vi "VM Spy - Dialog - Set Variable Value.vi"(6 "refresh writer ID":bool, 8 "writer ID in":u32, 9 "Display params":T1={"Num Format"=0, "Num Precision"=3, "Num Show I32"=FALSE, "Str Style"=0, "Str Wrap"=TRUE}, 10 "var name":string, 11 "VC Handle":T2=-1) -> (0 "Assigned":bool)   [LabVIEW 2021]
doc: "::: CalcExpress Toolkit :::\nCopyright (c) 2000-2026 Konstantin Shifershteyn. All rights reserved."
uses:
  vi.lib/addons/CalcExpress/cetypes.llb/VarMan Variable Context Handle.ctl
  <vilib>/Utility/miscctls.llb/LVKeyTypeDef.ctl
panel:
  in  "writer ID":u32
  in  "EnaWrap":bool=TRUE caption="Wrap"
  in  "int32":i32 caption="Int32" format="%.0x"
  in  "ShowInt32":bool caption="show I32"
  in  "IR":cluster{"Initial index":i32, "Final index":i32} caption="Index Range" {"Final index" min=0; "Initial index" min=0}
  in  "Format":u8(ring) items=["Floating point", "Scientific", "Engineering", "Binary", "Octal", "Hexadecimal", "Relative time", "Absolute time"]
  in  "prec":u8=2
  in  "a2str":string[][](array[string]) caption="Value"
  in  "a1str":string[](array[string]) caption="Value"
  in  "a2cdb":cdb[][](array[numeric]) caption="Value" format="%.2f"
  in  "a1cdb":cdb[](array[numeric]) caption="Value" format="%.2f"
  in  "cancel":bool
  in  "assign":bool
  in  "close":bool=TRUE caption="close window after assignment"
  in  "any":string
  in  "a2dbl":dbl[][](array[numeric]) caption="Value" format="%.2f"
  in  "cdb":cdb caption="Value" format="%.2f"
  in  "a1dbl":dbl[](array[numeric]) caption="Value" format="%.2f"
  in  "Display style":u32(ring) items=["Normal", "'\\' Code", "Password", "Hex dump"]
  in  "dbl":dbl caption="Value" format="%.3f"
  out "Context":string
  out "Variable":string
  in  "str":string caption="Value"
  # ":"
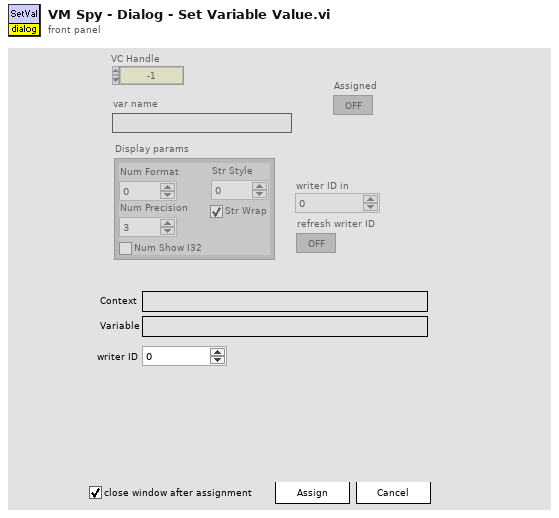
[diagram p1: front panel]
types:
  T1 = cluster{"Num Format":u32, "Num Precision":u32, "Num Show I32":bool, "Str Style":u32, "Str Wrap":bool}
  T2 = typedef "VarMan Variable Context Handle.ctl" = i32
  T3 = typedef "LVKeyTypeDef.ctl" = cluster{"Focus":bool, "Control":bool, "Shift":bool, "Key":string}
  T4 = enum32{"invalid app kind", "Development System", "Run Time System", "Student Edition", "Embedded LabVIEW", "Evaluation", "Custom"}
  T5 = typedef "eventvkey.ctl" = enum16{"ASCII", "Enter", "Return", "Shift", "Ctrl", "Alt", "Cmd", "Opt", "Caps", "NumLock", "Clear", "Break", "Up", "Down", "Left", "Right", "Insert", "Delete", "Home", "End", "PageUp", "PageDown", "Escape", "Help", "Pause", "ScrollLock", "F1", "F2", "F3", "F4", "F5", "F6", "F7", "F8", "F9", "F10", "F11", "F12", "F13", "F14", "F15", "F16", "F17", "F18", "F19", "F20", "F21", "F22", "F23", "F24", "Play", "VolumeUp", "VolumeDown", "Mute", "Two Byte Char"}
  T6 = cluster{"Shift":bool, "Ctrl":bool, "Alt":bool, "Cmd":bool, "Opt":bool}
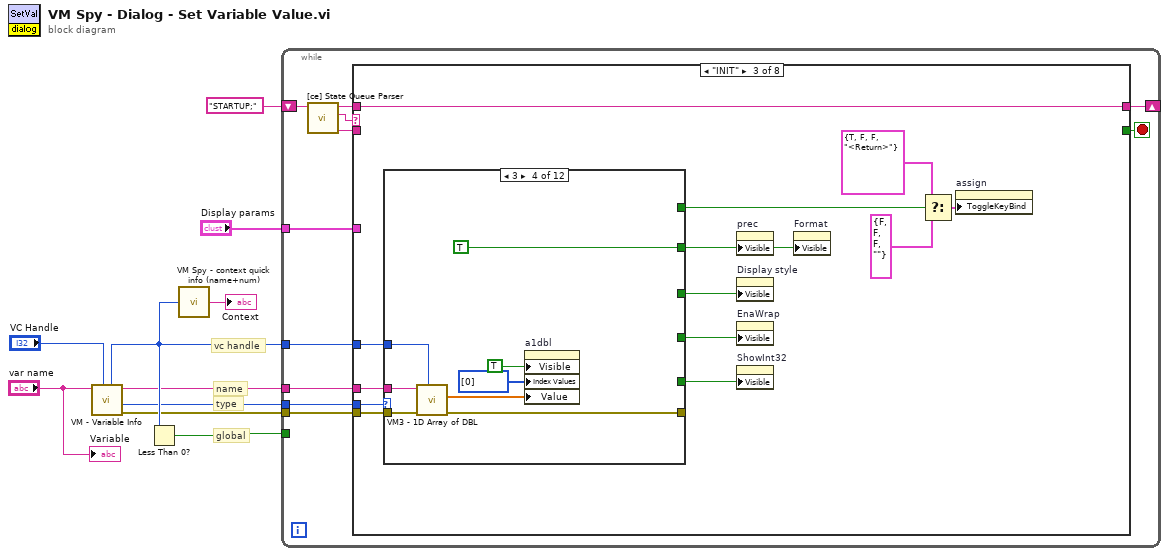
[diagram p0: block diagram]
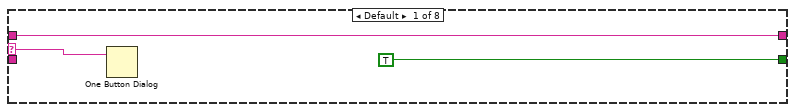
[diagram p2: hidden frame]
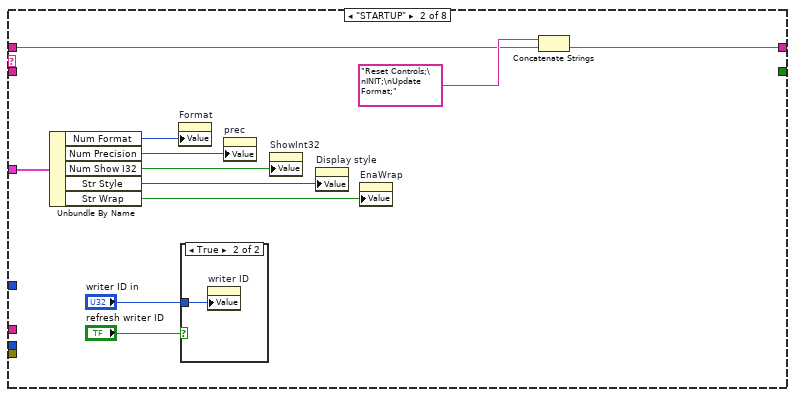
[diagram p3: hidden frame]
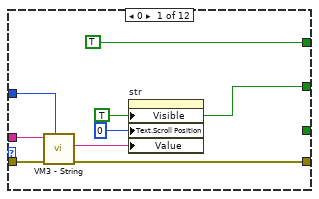
[diagram p5: hidden frame]
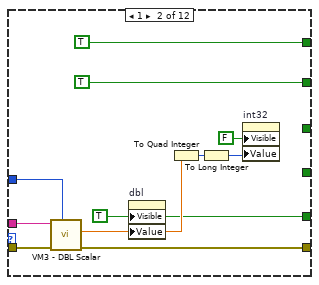
[diagram p6: hidden frame]
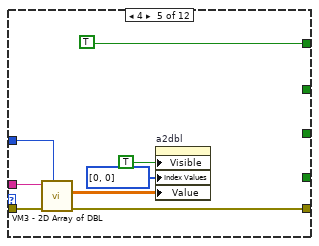
[diagram p8: hidden frame]
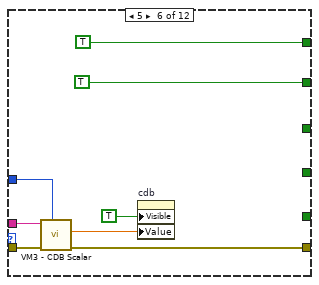
[diagram p9: hidden frame]
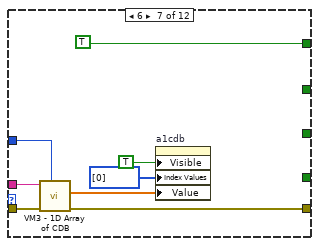
[diagram p10: hidden frame]
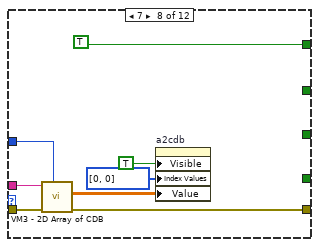
[diagram p11: hidden frame]
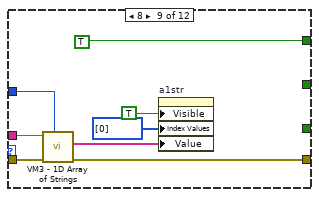
[diagram p12: hidden frame]
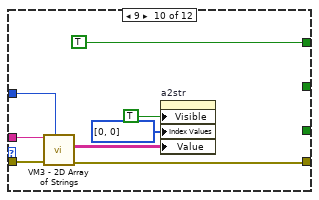
[diagram p13: hidden frame]
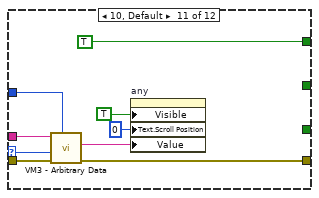
[diagram p14: hidden frame]
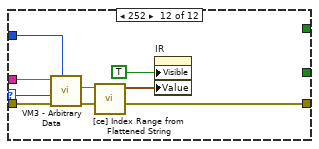
[diagram p15: hidden frame]
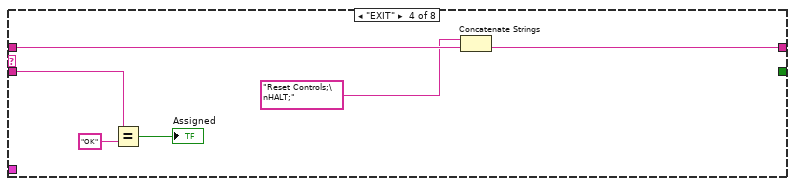
[diagram p16: hidden frame]
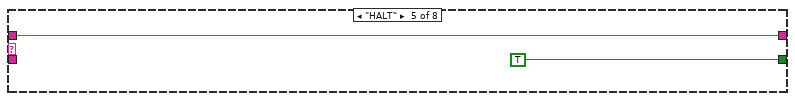
[diagram p17: hidden frame]
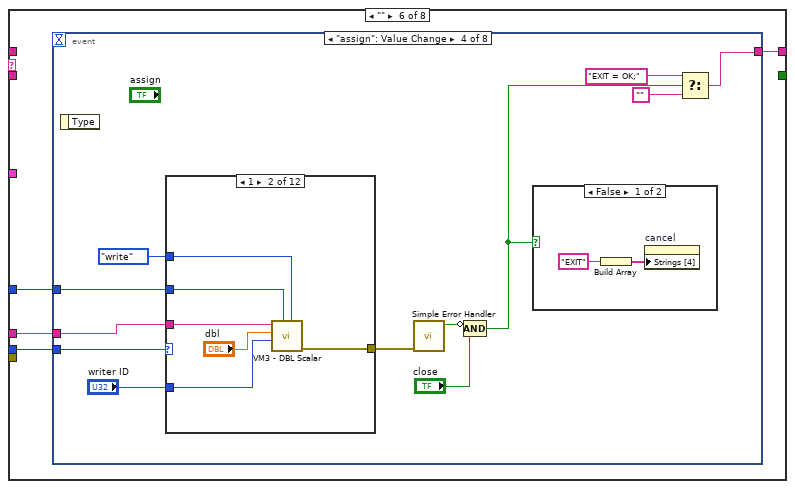
[diagram p18: hidden frame]
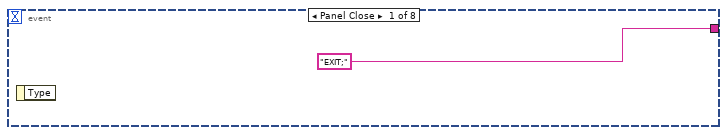
[diagram p19: hidden frame]
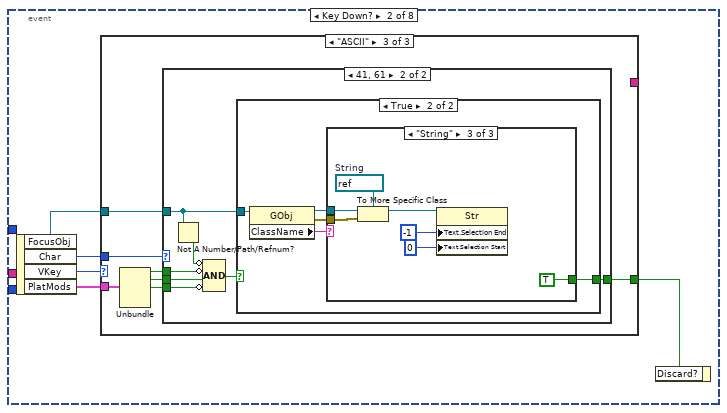
[diagram p20: hidden frame]
diagram:
  # "name"
  # "vc handle"
  # "type"
  # "global"
  n1 = call "VM - Variable Info.vi"("VC Handle"="VC Handle", "name_spec"="var name") -> ("error out"=w2:errorcluster, "var type"=w5:u32, "var name"=w7:string, "var VC Handle"=w8:T2)  [unwired: 4 in, 2 out]
  n2 = Less Than 0?(x=w8) -> (x < 0?=w6:bool)
  n3 = call "VM Spy - context quick info (name+num).vi"("handle"=w8) -> ("context info"=→"Context":string)  [unwired: 4 in]
  n4 = while {
    tunnel: w8 -> [w20]
    tunnel: w7 -> [w19]
    tunnel: w6 -> [_]
    tunnel: w5 -> [w18]
    shift-right: [w15] -> _
    shift-left: "STARTUP;" -> [w17]
    tunnel: w2 -> [w13]
    tunnel: "Display params" -> [w11]
    stop <- w21 stop-if-true
    n5 = call "[ce] State Queue Parser.vi"("input queue"=w17) -> ("state parameters"=w12:string, "state"=w16:string, "remained queue"=w14:string)  [unwired: 6 in]
    n6 = case shown="\"INIT\"" w16 {
      selector: w16 -> [w23 _ _ _ _ _ _ _]
      tunnel: [TRUE _ _ _ TRUE _ _ _] -> w21
      tunnel: w20 -> [_ _ w43 _ _ w154 _ _]
      tunnel: w19 -> [_ _ w42 _ _ w153 _ _]
      tunnel: w18 -> [_ _ w40 _ _ w152 _ w325]
      tunnel: [w24 w33 w39 w147 w150 w151 w317 w329] -> w15
      tunnel: w14 -> [w24 w34 w39 w148 w150 _ w317 w329]
      tunnel: w13 -> [_ _ w41 _ _ _ _ _]
      tunnel: w12 -> [_ _ _ w145 _ _ _ _]
      tunnel: w11 -> [_ w32 _ _ _ _ _ _]
      frame Default {
        n7 = One Button Dialog(message=w23) -> ()  [unwired: 1 in, 1 out]
      }
      frame "STARTUP" {
        n8 = Unbundle By Name(w32) -> ("Num Format"=w31:u32, "Num Precision"=w30:u32, "Num Show I32"=w29:bool, "Str Style"=w28:u32, "Str Wrap"=w27:bool)
        n9 = property on="Format" class="Ring (strict)"("Value"=w31) -> ()  [unwired: 2 in, 2 out]
        n10 = case shown="True" "refresh writer ID" {
          tunnel: "writer ID in" -> [_ w36]
          frame False {
          }
          frame True {
            n11 = property on="writer ID" class="DigNum (strict)"("Value"=w36) -> ()  [unwired: 2 in, 2 out]
          }
        }
        n12 = property on="prec" class="DigNum (strict)"("Value"=w30) -> ()  [unwired: 2 in, 2 out]
        n13 = property on="ShowInt32" class="Bool (strict)"("Value"=w29) -> ()  [unwired: 2 in, 2 out]
        n14 = property on="Display style" class="Ring (strict)"("Value"=w28) -> ()  [unwired: 2 in, 2 out]
        n15 = property on="EnaWrap" class="Bool (strict)"("Value"=w27) -> ()  [unwired: 2 in, 2 out]
        n16 = Concatenate Strings("Reset Controls;\nINIT;\nUpdate Format;" ("string"), w34) -> (w33:string)
      }
      frame "INIT" {
        n17 = case shown="3" w40 {
          selector: w40 -> [_ _ _ _ _ _ _ _ _ _ w130 w138]
          tunnel: w41 -> [w57 w67 w69 w76 w84 w92 w100 w108 w116 w124 w134 w142]
          tunnel: w42 -> [w56 w68 _ w77 w85 w93 w101 w109 w117 w125 w132 w140]
          tunnel: w43 -> [w54 w65 _ w74 w82 w90 w98 w106 w114 w122 w131 w139]
          tunnel: [w55 w66 w69 w75 w83 w91 w99 w107 w115 w123 w133 w141] -> _
          tunnel: [TRUE _ _ _ _ _ _ _ TRUE TRUE TRUE _] -> w49
          tunnel: [_ TRUE _ TRUE TRUE TRUE TRUE TRUE _ _ _ _] -> w48
          tunnel: [_ TRUE _ _ _ TRUE _ _ _ _ _ _] -> w44
          tunnel: [_ w59 _ _ _ _ _ _ _ _ _ _] -> w38
          tunnel: [w50 _ _ _ _ _ _ _ _ _ _ _] -> w37
          frame 0 {
            w50 = TRUE
            n18 = call "VM3 - String.vi"("VC Handle"=w54, "error in"=w57, "name_spec"=w56) -> ("error out"=w55:errorcluster, "value out"=w51:string)  [unwired: 5 in, 2 out]
            n19 = property on="str" class="Str"("Visible"=w50, "Text.Scroll Position"=u32 0, "Value"=w51) -> ()  [unwired: 2 in, 2 out]
          }
          frame 1 {
            w59 = TRUE
            n20 = call "VM3 - DBL Scalar.vi"("VC Handle"=w65, "error in"=w67, "name_spec"=w68) -> ("error out"=w66:errorcluster, "value out"=w62:dbl)  [unwired: 5 in, 2 out]
            n21 = property on="dbl" class="DigNum (strict)"("Visible"=w59, "Value"=w62) -> ()  [unwired: 2 in, 2 out]
            n22 = To Quad Integer(1:w62) -> (0:w61:i64)
            n23 = To Long Integer(number=w61) -> (32bit integer=w60:i32)
            n24 = property on="int32" class="DigNum (strict)"("Visible"=FALSE, "Value"=w60) -> ()  [unwired: 2 in, 2 out]
          }
          frame 2 {
          }
          frame 3 {
            n25 = call "VM3 - 1D Array of DBL.vi"("VC Handle"=w74, "error in"=w76, "name_spec"=w77) -> ("error out"=w75:errorcluster, "value out"=w70:dbl[])  [unwired: 5 in, 2 out]
            n26 = property on="a1dbl" class="Arr (strict)"("Visible"=TRUE, "Index Values"=u32[] [0], "Value"=w70) -> ()  [unwired: 2 in, 2 out]
          }
          frame 4 {
            n27 = call "VM3 - 2D Array of DBL.vi"("VC Handle"=w82, "error in"=w84, "name_spec"=w85) -> ("error out"=w83:errorcluster, "value out"=w78:dbl[][])  [unwired: 5 in, 2 out]
            n28 = property on="a2dbl" class="Arr (strict)"("Visible"=TRUE, "Index Values"=u32[] [0, 0], "Value"=w78) -> ()  [unwired: 2 in, 2 out]
          }
          frame 5 {
            n29 = call "VM3 - CDB Scalar.vi"("VC Handle"=w90, "error in"=w92, "name_spec"=w93) -> ("error out"=w91:errorcluster, "value out"=w86:cdb)  [unwired: 5 in, 2 out]
            n30 = property on="cdb" class="DigNum (strict)"("Visible"=TRUE, "Value"=w86) -> ()  [unwired: 2 in, 2 out]
          }
          frame 6 {
            n31 = call "VM3 - 1D Array of CDB.vi"("VC Handle"=w98, "error in"=w100, "name_spec"=w101) -> ("error out"=w99:errorcluster, "value out"=w94:cdb[])  [unwired: 5 in, 2 out]
            n32 = property on="a1cdb" class="Arr (strict)"("Visible"=TRUE, "Index Values"=u32[] [0], "Value"=w94) -> ()  [unwired: 2 in, 2 out]
          }
          frame 7 {
            n33 = call "VM3 - 2D Array of CDB.vi"("VC Handle"=w106, "error in"=w108, "name_spec"=w109) -> ("error out"=w107:errorcluster, "value out"=w102:cdb[][])  [unwired: 5 in, 2 out]
            n34 = property on="a2cdb" class="Arr (strict)"("Visible"=TRUE, "Index Values"=u32[] [0, 0], "Value"=w102) -> ()  [unwired: 2 in, 2 out]
          }
          frame 8 {
            n35 = call "VM3 - 1D Array of Strings.vi"("VC Handle"=w114, "error in"=w116, "name_spec"=w117) -> ("error out"=w115:errorcluster, "value out"=w110:string[])  [unwired: 5 in, 2 out]
            n36 = property on="a1str" class="Arr (strict)"("Visible"=TRUE, "Index Values"=u32[] [0], "Value"=w110) -> ()  [unwired: 2 in, 2 out]
          }
          frame 9 {
            n37 = call "VM3 - 2D Array of Strings.vi"("VC Handle"=w122, "error in"=w124, "name_spec"=w125) -> ("error out"=w123:errorcluster, "value out"=w118:string[][])  [unwired: 5 in, 2 out]
            n38 = property on="a2str" class="Arr (strict)"("Visible"=TRUE, "Index Values"=u32[] [0, 0], "Value"=w118) -> ()  [unwired: 2 in, 2 out]
          }
          frame 10, Default {
            n39 = call "VM3 - Arbitrary Data.vi"("var type in"=w130, "VC Handle"=w131, "error in"=w134, "name_spec"=w132) -> ("error out"=w133:errorcluster, "flattened value out"=w126:string)  [unwired: 3 in, 3 out]
            n40 = property on="any" class="Str"("Visible"=TRUE, "Text.Scroll Position"=u32 0, "Value"=w126) -> ()  [unwired: 2 in, 2 out]
          }
          frame 252 {
            n41 = call "VM3 - Arbitrary Data.vi"("var type in"=w138, "VC Handle"=w139, "error in"=w142, "name_spec"=w140) -> ("error out"=w141:errorcluster, "flattened value out"=w137:string)  [unwired: 3 in, 3 out]
            n42 = call "[ce] Index Range from Flattened String.vi"("Flattened string"=w137) -> ("Index Range"=w135:cluster{"Initial index":i32, "Final index":i32})  [unwired: 10 in]
            n43 = property on="IR" class="Clust (strict)"("Visible"=TRUE, "Value"=w135) -> ()  [unwired: 2 in, 2 out]
          }
        }
        n44 = property on="prec" class="DigNum (strict)"("Visible"=w48) -> ()  [unwired: 2 in, 2 out]
        n45 = property on="Display style" class="Ring (strict)"("Visible"=w49) -> ()  [unwired: 2 in, 2 out]
        n46 = property on="EnaWrap" class="Bool (strict)"("Visible"=w37) -> ()  [unwired: 2 in, 2 out]
        n47 = property on="ShowInt32" class="Bool (strict)"("Visible"=w38) -> ()  [unwired: 2 in, 2 out]
        n48 = property on="Format" class="Ring (strict)"("Visible"=w48) -> ()  [unwired: 2 in, 2 out]
        n49 = Select(t=T3 {"Focus"=TRUE, "Control"=FALSE, "Shift"=FALSE, "Key"="<Return>"} ("Toggle Key Binding"), s=w44, f=T3 {"Focus"=FALSE, "Control"=FALSE, "Shift"=FALSE, "Key"=""}) -> (s? t:f=w47:T3)
        n50 = property on="assign" class="Bool"("ToggleKeyBind"=w47) -> ()  [unwired: 2 in, 2 out]
      }
      frame "EXIT" {
        n51 = Equal?(x=w145, y="OK") -> (x = y?=→"Assigned":bool)
        n52 = Concatenate Strings("Reset Controls;\nHALT;" ("string"), w148) -> (w147:string)
      }
      frame "HALT" {
      }
      frame "" {
        n53 = event shown="[3] \"assign\": Value Change" {
          selector: _ -> [_ _ _ _ _ _ _ _]
          dyn-events: _ -> [_ _ _ _ _ _ _ _]
          timeout: _ -> [_ _ _ _ _ _ _ _]
          tunnel: w154 -> [_ _ _ w219 _ _ _ _]
          tunnel: w153 -> [_ _ _ w218 _ _ _ _]
          tunnel: w152 -> [_ _ _ w217 _ _ _ _]
          tunnel: ["EXIT;" _ "EXIT;" w214 "Update Format;" "Update Format;" _ _] -> w151
          event Panel Close {
            n54 = event-data() -> ()  [unwired: 1 in, 1 out]
          }
          event Key Down? {
            n55 = event-data() -> ("FocusObj"=w157:refnum<vi>, "Char"=w158:i16, "VKey"=w159:T5, "PlatMods"=w160:T6)  [unwired: 1 in]
            n56 = case shown="\"ASCII\"" w159 {
              tunnel: w160 -> [_ w176 w183]
              tunnel: [_ w162 w177] -> w156
              tunnel: [_ w170 _] -> _
              tunnel: w158 -> [_ _ w179]
              tunnel: w157 -> [_ _ w178]
              frame Default {
              }
              frame "Escape" {
                n57 = Current VI's Path() -> (path=w169:path)
                n58 = property class="App"() -> ("App.Kind"=w167:T4, "App.Dir"=w168:path)  [unwired: 2 in, 2 out]
                n59 = Unbundle(w176) -> ("Shift"=w175:bool, "Ctrl"=w174:bool, "Alt"=w173:bool)  [unwired: 2 out]
                n60 = Compound Arithmetic op=AND(w175, invert w174, invert w173) -> (w162:bool)
                n61 = call <vilib>:"Compare Two Paths.vi"("Path 2"=w169, "Path 1"=w168) -> ("Path 2 Relative to Path 1?"=w165:bool)  [unwired: 6 in, 3 out]
                n62 = Not Equal?(x=T4."Development System", y=w167) -> (x != y?=w166:bool)
                n63 = Not Or(1:w165, 2:w166) -> (0:w164:bool)
                n64 = And(x=w164, y=w162) -> (x .and. y?=w161:bool)
                n65 = Select(t="EXIT = KeepFPOpen;", s=w161, f="") -> (s? t:f=w170:string)
              }
              frame "ASCII" {
                n66 = Unbundle(w183) -> ("Shift"=w182:bool, "Ctrl"=w181:bool, "Alt"=w180:bool)  [unwired: 2 out]
                n67 = case shown="41, 61" w179 {
                  tunnel: w182 -> [_ w190]
                  tunnel: w181 -> [_ w189]
                  tunnel: w180 -> [_ w188]
                  tunnel: w178 -> [_ w185]
                  tunnel: [_ w184] -> w177
                  frame Default {
                  }
                  frame 65, 97 {
                    n68 = Not A Number/Path/Refnum?(number/path/refnum=w185) -> (NaN/Path/Refnum?=w187:bool)
                    n69 = Compound Arithmetic op=AND(invert w187, invert w190, w189, invert w188) -> (w186:bool)
                    n70 = case shown="True" w186 {
                      tunnel: w185 -> [_ w195]
                      tunnel: [_ w193] -> w184
                      frame False {
                      }
                      frame True {
                        n71 = property class="GObj"(reference=w195) -> (reference out=w192:refnum<vi>, error out=w191:errorcluster, "ClassName"=w194:string)  [unwired: 1 in]
                        n72 = case shown="\"String\"" w194 {
                          tunnel: [_ TRUE TRUE] -> w193
                          tunnel: w192 -> [_ w200 w207]
                          tunnel: w191 -> [_ w199 w206]
                          frame Default {
                          }
                          frame "Digital" {
                            w201 = refnum<vi> refnum  # Digital
                            n73 = To More Specific Class(target class=w201, reference=w200, error in=w199) -> (specific class reference=w198:refnum<vi>)  [unwired: 1 out]
                            n74 = property class="DigNum"(reference=w198, "NumText.Selection End"=-1 ("Numeric Text.Selection:End"), "NumText.Selection Start"=u32 0 ("Numeric Text.Selection:Start")) -> ()  [unwired: 1 in, 2 out]
                          }
                          frame "String" {
                            w208 = refnum<vi> refnum  # String
                            n75 = To More Specific Class(target class=w208, reference=w207, error in=w206) -> (specific class reference=w205:refnum<vi>)  [unwired: 1 out]
                            n76 = property class="Str"(reference=w205, "Text.Selection End"=-1 ("Numeric Text.Selection:End"), "Text.Selection Start"=u32 0 ("Numeric Text.Selection:Start")) -> ()  [unwired: 1 in, 2 out]
                          }
                        }
                      }
                    }
                  }
                }
              }
            }
            n77 = event-data("Discard?"=w156) -> ()  [unwired: 1 in, 1 out]
          }
          event "cancel": Value Change {
            n78 = event-data() -> ()  [unwired: 1 in, 1 out]
          }
          event "assign": Value Change {
            n79 = event-data() -> ()  [unwired: 1 in, 1 out]
            n80 = case shown="1" w217 {
              selector: w217 -> [_ _ _ _ _ _ _ _ _ _ w282 w291]
              tunnel: w218 -> [w230 w236 _ w242 w248 w254 w260 w266 w272 w278 w285 w293]
              tunnel: w219 -> [w227 w235 _ w239 w245 w251 w257 w263 w269 w275 w284 w292]
              tunnel: [w228 w233 _ w240 w247 w253 w259 w265 w271 w277 w281 w290] -> w220
              tunnel: enum16{"create", "destroy", "write", "read"}."write" ("cmd (read)") -> [w226 w232 _ w238 w244 w250 w256 w261 w268 w273 w280 w287]
              tunnel: "writer ID" -> [w225 w231 _ w237 w243 w249 w255 w262 w267 w274 w279 w286]
              frame 0 {
                n81 = call "VM3 - String.vi"("cmd (read)"=w226, "VC Handle"=w227, "writer ID"=w225, "value in"="str", "name_spec"=w230) -> ("error out"=w228:errorcluster)  [unwired: 3 in, 3 out]
              }
              frame 1 {
                n82 = call "VM3 - DBL Scalar.vi"("cmd (read)"=w232, "VC Handle"=w235, "writer ID"=w231, "value in"="dbl", "name_spec"=w236) -> ("error out"=w233:errorcluster)  [unwired: 3 in, 3 out]
              }
              frame 2 {
              }
              frame 3 {
                n83 = call "VM3 - 1D Array of DBL.vi"("cmd (read)"=w238, "VC Handle"=w239, "writer ID"=w237, "value in"="a1dbl", "name_spec"=w242) -> ("error out"=w240:errorcluster)  [unwired: 3 in, 3 out]
              }
              frame 4 {
                n84 = call "VM3 - 2D Array of DBL.vi"("cmd (read)"=w244, "VC Handle"=w245, "writer ID"=w243, "value in"="a2dbl", "name_spec"=w248) -> ("error out"=w247:errorcluster)  [unwired: 3 in, 3 out]
              }
              frame 5 {
                n85 = call "VM3 - CDB Scalar.vi"("cmd (read)"=w250, "VC Handle"=w251, "writer ID"=w249, "value in"="cdb", "name_spec"=w254) -> ("error out"=w253:errorcluster)  [unwired: 3 in, 3 out]
              }
              frame 6 {
                n86 = call "VM3 - 1D Array of CDB.vi"("cmd (read)"=w256, "VC Handle"=w257, "writer ID"=w255, "value in"="a1cdb", "name_spec"=w260) -> ("error out"=w259:errorcluster)  [unwired: 3 in, 3 out]
              }
              frame 7 {
                n87 = call "VM3 - 2D Array of CDB.vi"("cmd (read)"=w261, "VC Handle"=w263, "writer ID"=w262, "value in"="a2cdb", "name_spec"=w266) -> ("error out"=w265:errorcluster)  [unwired: 3 in, 3 out]
              }
              frame 8 {
                n88 = call "VM3 - 1D Array of Strings.vi"("cmd (read)"=w268, "VC Handle"=w269, "writer ID"=w267, "value in"="a1str", "name_spec"=w272) -> ("error out"=w271:errorcluster)  [unwired: 3 in, 3 out]
              }
              frame 9 {
                n89 = call "VM3 - 2D Array of Strings.vi"("cmd (read)"=w273, "VC Handle"=w275, "writer ID"=w274, "value in"="a2str", "name_spec"=w278) -> ("error out"=w277:errorcluster)  [unwired: 3 in, 3 out]
              }
              frame 10, Default {
                n90 = call "VM3 - Arbitrary Data.vi"("cmd (read)"=w280, "var type in"=w282, "VC Handle"=w284, "writer ID"=w279, "flattened value in"="any", "name_spec"=w285) -> ("error out"=w281:errorcluster)  [unwired: 1 in, 4 out]
              }
              frame 252 {
                n91 = call "[ce] Index Range to Flattened String.vi"("Index Range"="IR") -> ("Flattened string"=w288:string)  [unwired: 10 in]
                n92 = call "VM3 - Arbitrary Data.vi"("cmd (read)"=w287, "var type in"=w291, "VC Handle"=w292, "writer ID"=w286, "flattened value in"=w288, "name_spec"=w293) -> ("error out"=w290:errorcluster)  [unwired: 1 in, 4 out]
              }
            }
            n93 = call <vilib>:"Simple Error Handler.vi"("error in (no error)"=w220) -> ("error?"=w222:bool)  [unwired: 4 in, 4 out]
            n94 = Compound Arithmetic op=AND(invert w222, "close") -> (w211:bool)
            n95 = case shown="False" w211 {
              frame False {
                n96 = Build Array("EXIT") -> (w224:string[])
                n97 = property on="cancel" class="Bool"("Strings [4]"=w224) -> ()  [unwired: 2 in, 2 out]
              }
              frame True {
              }
            }
            n98 = Select(t="EXIT = OK;", s=w211, f="") -> (s? t:f=w214:string)
          }
          event "Format", "prec", "Display style", "EnaWrap": Value Change {
            n99 = event-data() -> ()  [unwired: 1 in, 1 out]
          }
          event "ShowInt32": Value Change {
            n100 = event-data() -> ()  [unwired: 1 in, 1 out]
          }
          event "dbl": Value Change {
            n101 = event-data() -> ("NewVal"=w297:dbl)  [unwired: 1 in, 2 out]
            n102 = To Quad Integer(1:w297) -> (0:w298:i64)
            n103 = To Long Integer(number=w298) -> (32bit integer=w296:i32)
            n104 = property on="int32" class="DigNum (strict)"("Value"=w296) -> ()  [unwired: 2 in, 2 out]
          }
          event "int32": Value Change {
            n105 = event-data() -> ("NewVal"=w300:i32)  [unwired: 1 in]
            n106 = To Double Precision Float(number=w300) -> (double precision float=w299:dbl)
            n107 = property on="dbl" class="DigNum (strict)"("Value"=w299) -> ()  [unwired: 2 in, 2 out]
          }
        }
      }
      frame "Reset Controls" {
        w304 = FALSE ("Visible")
        n108 = control-ref of="IR"() -> (w306:refnum<vi>)
        n109 = control-ref of="dbl"() -> (w316:refnum<vi>)
        n110 = control-ref of="cdb"() -> (w313:refnum<vi>)
        n111 = control-ref of="str"() -> (w310:refnum<vi>)
        n112 = control-ref of="any"() -> (w307:refnum<vi>)
        n113 = control-ref of="int32"() -> (w303:refnum<vi>)
        n114 = control-ref of="a1dbl"() -> (w315:refnum<vi>)
        n115 = control-ref of="a2dbl"() -> (w314:refnum<vi>)
        n116 = control-ref of="a1cdb"() -> (w312:refnum<vi>)
        n117 = control-ref of="a2cdb"() -> (w311:refnum<vi>)
        n118 = control-ref of="a1str"() -> (w309:refnum<vi>)
        n119 = control-ref of="a2str"() -> (w308:refnum<vi>)
        n120 = Build Array(w316, w315, w314, w313, w312, w311, w310, w309, w308, w307, w306, w303) -> (w305:refnum<vi>[])
        n121 = property on="prec" class="DigNum (strict)"("Visible"=w304) -> ()  [unwired: 2 in, 2 out]
        n122 = for {
          tunnel: w305 -> [w320] mode=indexing
          n123 = property class="Ctl"(reference=w320, "Visible"=FALSE) -> (reference out=w318:refnum<vi>)  [unwired: 1 in, 1 out]
          n124 = invoke class="Ctl" method="Reinit To Default"(reference=w318) -> ()  [unwired: 2 in, 3 out]
        }
        n125 = Build Array("Cancel") -> (w302:string[])
        n126 = property on="Format" class="Ring (strict)"("Visible"=w304) -> ()  [unwired: 2 in, 2 out]
        n127 = property on="cancel" class="Bool"("Strings [4]"=w302) -> ()  [unwired: 2 in, 2 out]
        n128 = property on="Display style" class="Ring (strict)"("Visible"=w304) -> ()  [unwired: 2 in, 2 out]
        n129 = property on="EnaWrap" class="Bool (strict)"("Visible"=w304) -> ()  [unwired: 2 in, 2 out]
        n130 = property on="ShowInt32" class="Bool (strict)"("Visible"=w304) -> ()  [unwired: 2 in, 2 out]
      }
      frame "Update Format" {
        n131 = property on="ShowInt32" class="Bool (strict)"() -> ("Visible"=w323:bool, "Value"=w322:bool)  [unwired: 2 in, 2 out]
        n132 = case shown="1" w325 {
          tunnel: "Display style" -> [w332 _ _ _ _ _ _ _ w345 w346 w347 _]
          tunnel: "Format" -> [_ w334 _ w336 w338 w340 w342 w344 _ _ _ _]
          tunnel: "prec" -> [_ w333 _ w335 w337 w339 w341 w343 _ _ _ _]
          tunnel: "EnaWrap" -> [w330 _ _ _ _ _ _ _ _ _ _ _]
          frame 0 {
            n133 = Not(x=w330) -> (.not. x?=w331:bool)
            n134 = property on="str" class="Str"("Display Style"=w332, "WrappingEnabled"=w330, "HScrollVis"=w331) -> ()  [unwired: 2 in, 2 out]
          }
          frame 1 {
            n135 = property on="dbl" class="DigNum (strict)"("Display Format:Format"=w334, "Display Format:Precision"=w333) -> ()  [unwired: 2 in, 2 out]
          }
          frame 2 {
          }
          frame 3 {
            n136 = property on="dbl" class="DigNum (strict)"("Display Format:Format"=w336, "Display Format:Precision"=w335) -> ()  [unwired: 2 in, 2 out]
          }
          frame 4 {
            n137 = property on="dbl" class="DigNum (strict)"("Display Format:Format"=w338, "Display Format:Precision"=w337) -> ()  [unwired: 2 in, 2 out]
          }
          frame 5 {
            n138 = property on="cdb" class="DigNum (strict)"("Display Format:Format"=w340, "Display Format:Precision"=w339) -> ()  [unwired: 2 in, 2 out]
          }
          frame 6 {
            n139 = property on="dbl" class="DigNum (strict)"("Display Format:Format"=w342, "Display Format:Precision"=w341) -> ()  [unwired: 2 in, 2 out]
          }
          frame 7 {
            n140 = property on="dbl" class="DigNum (strict)"("Display Format:Format"=w344, "Display Format:Precision"=w343) -> ()  [unwired: 2 in, 2 out]
          }
          frame 8 {
            n141 = property class="Str"("Display Style"=w345) -> ()  [unwired: 2 in, 2 out]
          }
          frame 9 {
            n142 = property class="Str"("Display Style"=w346) -> ()  [unwired: 2 in, 2 out]
          }
          frame 10, Default {
            n143 = property on="any" class="Str"("Display Style"=w347) -> ()  [unwired: 2 in, 2 out]
          }
          frame 252 {
          }
        }
        n144 = And(x=w323, y=w322) -> (x .and. y?=w321:bool)
        n145 = property on="int32" class="DigNum (strict)"("Visible"=w321) -> ()  [unwired: 2 in, 2 out]
      }
    }
  }
  "Variable" <- "var name"
